vi "project.Industrial_Control.vi"() -> ()   [LabVIEW 2020]
doc: "ASTRA educational industrial automation simulation. Six-tab HMI; role-based authentication; conveyor state machine; deterministic sensors; alarm lifecycle; CSV journal. Logout/timeout/Exit request a controlled stop. No physical I/O or certified safety function. See docs/Engineering_Report.pdf and TEST_RESULTS.md. Public demonstration credentials only."
panel:
  out "Access level":string="None"
  out "Current operator":string="None"
  out "Authentication status":string="Signed out - enter your credentials"
  in  "Navigation":T1(tab)
  out "Can administer":bool
  out "Can acknowledge or reset":bool
  out "Can start or stop":bool
  out "Account lockout remaining (s)":dbl
  in  "Logout":bool
  in  "Username":string
  in  "Password":string
  in  "Login":bool
  out "Authenticated":bool
  out "Failed attempts":dbl
  out "Motor current (A)":dbl
  out "Motor temperature (C)":dbl=25.0 caption="Motor temperature (°C)"
  in  "Start conveyor":bool
  in  "Stop conveyor":bool
  out "Machine state":T2(ring)
  out "Operating mode":string="SOFTWARE SIMULATION"
  out "Motor speed (RPM)":dbl(knob) scale=0.0..1500.0
  out "Motor running":bool
  out "Motor stopped":bool=TRUE
  out "Machine fault":bool
  out "Machine message":string="Initializing"
  out "Sensor quality":string="GOOD"
  out "Monitoring trip":bool
  out "Current warning":bool
  out "Temperature warning":bool
  out "Sensor data valid":bool=TRUE
  out "Active current trip (A)":dbl=9.0
  out "Active current warning (A)":dbl=6.0
  out "Active temperature trip (C)":dbl=90.0 caption="Active temperature trip (°C)"
  out "Active temperature warning (C)":dbl=75.0 caption="Active temperature warning (°C)"
  out "Monitored speed (RPM)":dbl
  out "Current (A)":dbl(knob) scale=0.0..16.0
  out "Temperature (C)":dbl(knob)=25.0 caption="Temperature (°C)" scale=0.0..120.0
  out "Alarm history":string
  out "Unacknowledged alarms":dbl
  out "Active alarm severity":string="NORMAL"
  in  "Acknowledge all alarms":bool
  out "Alarm register":string[][](table)
  in  "Reset fault":bool
  out "Audit history":string
  out "CSV log path":path=path "logs/events.csv"
  in  "Inject sensor failure":bool
  in  "Inject overtemperature":bool
  in  "Apply monitoring settings":bool
  in  "Current trip setpoint (A)":dbl=9.0
  in  "Current warning setpoint (A)":dbl=6.0
  in  "Temperature trip setpoint (C)":dbl=90.0 caption="Temperature trip setpoint (°C)"
  in  "Temperature warning setpoint (C)":dbl=75.0 caption="Temperature warning setpoint (°C)"
  in  "Start permissive healthy":bool=TRUE
  in  "Inject motor overload":bool
  in  "Inject drive fault":bool
  in  "Generate demo password":bool
  out "Generated demonstration password":string
  out "Settings result":string="Default thresholds active"
  out "Session remaining (s)":dbl
  out "Audit write healthy":bool=TRUE
  in  "Exit application":bool
  # "INDUSTRIAL CONTROL & MONITORING"
  # "Credentials are case-sensitive. Three failures lock that account for 30 seconds."
  # "Use the demonstration account details in README.md. Logout before changing users."
  # "Logout / timeout: controlled stop. Fault reset: Maintenance or Administrator."
  # "Only Administrators can change simulation inputs and thresholds."
  # "ADMINISTRATOR UTILITY"
  # "This utility does not create, replace or reveal an authentication password."
  # "Ordinary random numbers are not cryptographically secure. Output is never logged."
  # "The original ten-iteration For Loop is retained with corrected digit conversion."
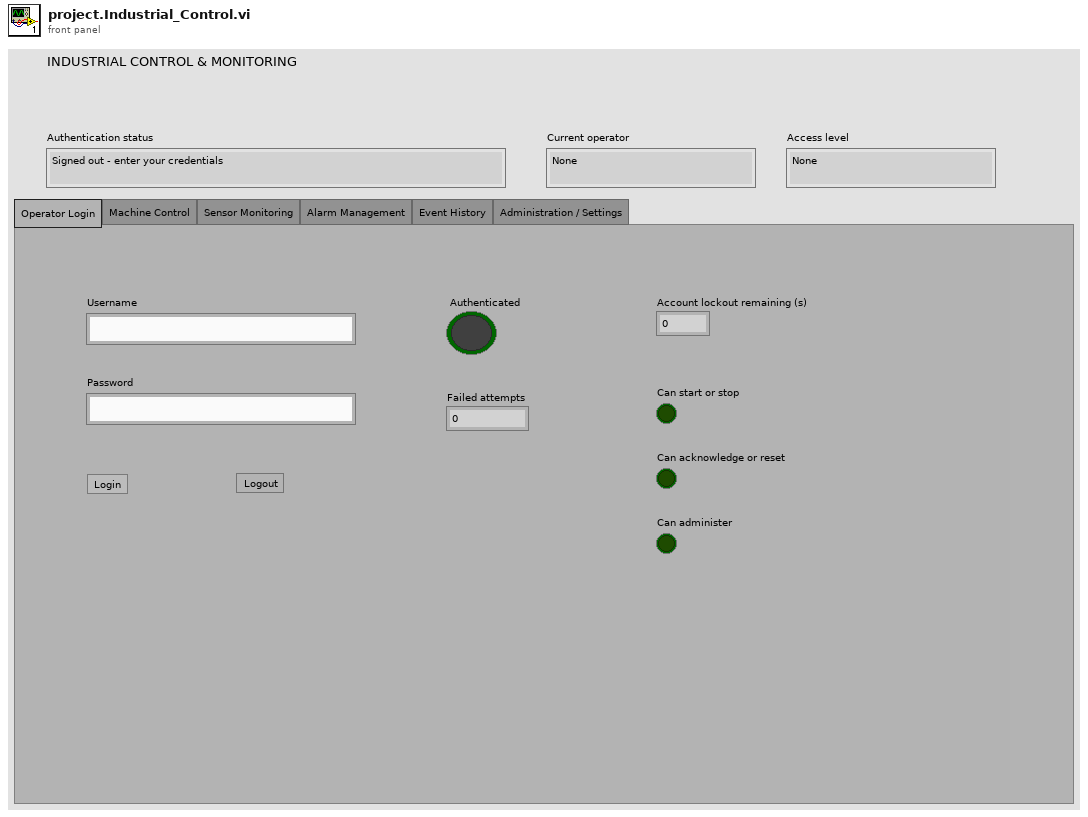
[diagram p1: front panel]
types:
  T1 = enum32{"Operator Login", "Machine Control", "Sensor Monitoring", "Alarm Management", "Event History", "Administration / Settings"}
  T2 = enum16{"INITIALIZATION", "IDLE", "READY", "RUNNING", "STOPPING", "FAULT", "RESETTING"}
  T3 = cluster{"A101":string, "A102":string, "A103":string, "A104":string, "A105":string, "A106":string, "A107":string, "A108":string, "A109":string}
  T4 = cluster{"A101 Active":dbl, "A101 Acknowledged":dbl, "A101 Seen":dbl, "A101 Changed":dbl, "A102 Active":dbl, "A102 Acknowledged":dbl, "A102 Seen":dbl, "A102 Changed":dbl, "A103 Active":dbl, "A103 Acknowledged":dbl, "A103 Seen":dbl, "A103 Changed":dbl, "A104 Active":dbl, "A104 Acknowledged":dbl, "A104 Seen":dbl, "A104 Changed":dbl, "A105 Active":dbl, "A105 Acknowledged":dbl, "A105 Seen":dbl, "A105 Changed":dbl, "A106 Active":dbl, "A106 Acknowledged":dbl, "A106 Seen":dbl, "A106 Changed":dbl, "A107 Active":dbl, "A107 Acknowledged":dbl, "A107 Seen":dbl, "A107 Changed":dbl, "A108 Active":dbl, "A108 Acknowledged":dbl, "A108 Seen":dbl, "A108 Changed":dbl, "A109 Active":dbl, "A109 Acknowledged":dbl, "A109 Seen":dbl, "A109 Changed":dbl}
  T5 = cluster{"Temperature C":dbl, "Current A":dbl, "Previous tick ms":dbl, "Temperature warning C":dbl, "Temperature trip C":dbl, "Current warning A":dbl, "Current trip A":dbl, "Settings result":dbl}
  T6 = cluster{"Machine state":enum16{"INITIALIZATION", "IDLE", "READY", "RUNNING", "STOPPING", "FAULT", "RESETTING"}, "Speed RPM":dbl, "Previous tick ms":dbl, "Reset started ms":dbl, "Latched fault code":dbl, "Command result":dbl, "Transition sequence":dbl}
  T7 = cluster{"Operator failures":dbl, "Maintenance failures":dbl, "Administrator failures":dbl, "Operator lock start ms":dbl, "Maintenance lock start ms":dbl, "Administrator lock start ms":dbl, "Active account":dbl, "Last activity ms":dbl, "Status code":dbl, "Event sequence":dbl}
  T8 = cluster{"Machine state":enum16{"INITIALIZATION", "IDLE", "READY", "RUNNING", "STOPPING", "FAULT", "RESETTING"}, "Speed RPM":dbl, i16, i16, i16, i16, i16, "Temperature warning setpoint (C)":dbl, "Temperature trip setpoint (C)":dbl, "Current warning setpoint (A)":dbl, "Current trip setpoint (A)":dbl}
  T9 = cluster{"High temperature warning":dbl, "Overtemperature trip":dbl, "High current warning":dbl, "Overload trip":dbl, "Sensor failure":dbl}
  T10 = cluster{"High temperature warning":dbl, "Overtemperature trip":dbl, "High current warning":dbl, "Overload trip":dbl, "Sensor failure":dbl, "unauthorized":dbl, "locked":dbl, i16, "permit_alarm":dbl}
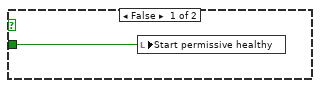
[diagram p2: hidden frame]
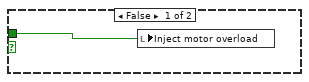
[diagram p3: hidden frame]
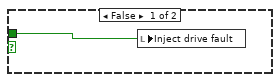
[diagram p4: hidden frame]
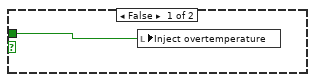
[diagram p5: hidden frame]
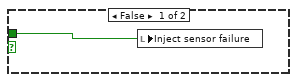
[diagram p6: hidden frame]
diagram:
  n1 = control-ref of="This VI"() -> (w23:refnum<vi>)
  n2 = property class="VI"(reference=w23) -> ("Path"=w22:path)  [unwired: 1 in, 2 out]
  n3 = Strip Path(path=w22) -> (stripped path=w21:path)  [unwired: 1 out]
  n4 = Build Path(base path=w21, name or relative path="logs\\events.csv") -> (appended path=w19:path)
  n5 = while {
    shift-right: [w446] -> _
    shift-left: T7 {"Operator failures"=0.0, "Maintenance failures"=0.0, "Administrator failures"=0.0, "Operator lock start ms"=-1.0, "Maintenance lock start ms"=-1.0, "Administrator lock start ms"=-1.0, "Active account"=-1.0, "Last activity ms"=0.0, "Status code"=0.0, "Event sequence"=0.0} ("State in") -> [w445]
    shift-right: ["Username"] -> _
    shift-left: "" -> [w439]
    shift-right: ["Password"] -> _
    shift-left: "" -> [w438]
    shift-right: ["Navigation"] -> _
    shift-left: 0 -> [w434]
    shift-right: [w390] -> _
    shift-left: "" -> [w391]
    tunnel: w19 -> [w382]
    tunnel: w19 -> [_]
    shift-right: [w381] -> _
    shift-left: "" -> [w380]
    shift-right: [w379] -> _
    shift-left: TRUE -> [w378]
    shift-right: [w377] -> _
    shift-left: T6 {"Machine state"=enum."INITIALIZATION", "Speed RPM"=0.0, "Previous tick ms"=-1.0, "Reset started ms"=-1.0, "Latched fault code"=0.0, "Command result"=0.0, "Transition sequence"=0.0} ("State in") -> [w376]
    shift-right: [w371] -> _
    shift-left: FALSE -> [w372]
    shift-right: [w29] -> _
    shift-left: TRUE -> [w359]
    shift-right: [w30] -> _
    shift-left: FALSE -> [w354]
    shift-right: [w31] -> _
    shift-left: FALSE -> [w349]
    shift-right: ["Start permissive healthy"] -> _
    shift-left: TRUE -> [w332]
    shift-right: ["Inject motor overload"] -> _
    shift-left: FALSE -> [w329]
    shift-right: ["Inject drive fault"] -> _
    shift-left: FALSE -> [w326]
    shift-right: [w32] -> _
    shift-left: FALSE -> [w274]
    shift-right: [w33] -> _
    shift-left: FALSE -> [w269]
    shift-right: [w247] -> _
    shift-left: T5 {"Temperature C"=25.0, "Current A"=0.0, "Previous tick ms"=-1.0, "Temperature warning C"=75.0, "Temperature trip C"=90.0, "Current warning A"=6.0, "Current trip A"=9.0, "Settings result"=0.0} ("State in") -> [w246]
    shift-right: [w188] -> _
    shift-left: T4 {"A101 Active"=0.0, "A101 Acknowledged"=1.0, "A101 Seen"=0.0, "A101 Changed"=0.0, "A102 Active"=0.0, "A102 Acknowledged"=1.0, "A102 Seen"=0.0, "A102 Changed"=0.0, "A103 Active"=0.0, "A103 Acknowledged"=1.0, "A103 Seen"=0.0, "A103 Changed"=0.0, "A104 Active"=0.0, "A104 Acknowledged"=1.0, "A104 Seen"=0.0, "A104 Changed"=0.0, "A105 Active"=0.0, "A105 Acknowledged"=1.0, "A105 Seen"=0.0, "A105 Changed"=0.0, "A106 Active"=0.0, "A106 Acknowledged"=1.0, "A106 Seen"=0.0, "A106 Changed"=0.0, "A107 Active"=0.0, "A107 Acknowledged"=1.0, "A107 Seen"=0.0, "A107 Changed"=0.0, "A108 Active"=0.0, "A108 Acknowledged"=1.0, "A108 Seen"=0.0, "A108 Changed"=0.0, "A109 Active"=0.0, "A109 Acknowledged"=1.0, "A109 Seen"=0.0, "A109 Changed"=0.0} ("State in") -> [w187]
    shift-right: [w158] -> _
    shift-left: T3 {"A101"="", "A102"="", "A103"="", "A104"="", "A105"="", "A106"="", "A107"="", "A108"="", "A109"=""} ("Previous timestamps") -> [w157]
    shift-right: [w149] -> _
    shift-left: "" -> [w151]
    shift-right: ["Inject overtemperature"] -> _
    shift-left: FALSE -> [w49]
    shift-right: ["Inject sensor failure"] -> _
    shift-left: FALSE -> [w46]
    stop <- w333 stop-if-true
    w115 = ""
    (unwired) "\t"
    w162 = "system"
    n6 = Wait (ms)(milliseconds to wait=50) -> ()  [unwired: 1 out]
    n7 = Select(t=1, s="Start conveyor", f=0) -> (s? t:f=w364:i32)
    n8 = Select(t=3, s="Reset fault", f=w364) -> (s? t:f=w361:i32)
    n9 = Select(t=3, s="Generate demo password", f=0) -> (s? t:f=w452:i32)
    n10 = Select(t=2, s="Stop conveyor", f=w361) -> (s? t:f=w340:i32)
    n11 = Not Equal?(x=w439, y="Username") -> (x != y?=w437:bool)
    n12 = Not Equal?(x=w438, y="Password") -> (x != y?=w436:bool)
    n13 = call "Final Demo Credential Lookup.vi"("Password"="Password", "Username"="Username") -> ("Credentials match"=w460:bool, "Account index"=w461:dbl)  [unwired: 8 in]
    n14 = Not Equal?(x=w332, y="Start permissive healthy") -> (x != y?=w330:bool)
    n15 = Or(x="Exit application", y="Logout") -> (x .or. y?=w450:bool)
    n16 = Not Equal To 0?(x=w340) -> (x != 0?=w331:bool)
    n17 = Select(t=1, s="Login", f=w452) -> (s? t:f=w448:i32)
    n18 = Or(x=w331, y=w330) -> (x .or. y?=w328:bool)
    n19 = Or(x=w436, y=w437) -> (x .or. y?=w433:bool)
    n20 = Not Equal?(x=w434, y="Navigation") -> (x != y?=w432:bool)
    n21 = Not Equal?(x=w329, y="Inject motor overload") -> (x != y?=w327:bool)
    n22 = Select(t=2, s=w450, f=w448) -> (s? t:f=w447:i32)
    n23 = Or(x=w328, y=w327) -> (x .or. y?=w325:bool)
    n24 = Or(x=w432, y=w433) -> (x .or. y?=w431:bool)
    n25 = Not Equal?(x=w326, y="Inject drive fault") -> (x != y?=w324:bool)
    n26 = Or(x="Acknowledge all alarms", y="Apply monitoring settings") -> (x .or. y?=w48:bool)
    n27 = Not Equal?(x=w49, y="Inject overtemperature") -> (x != y?=w47:bool)
    n28 = Not Equal To 0?(x=w447) -> (x != 0?=w430:bool)
    n29 = Or(x=w325, y=w324) -> (x .or. y?=w322:bool)
    n30 = Or(x=w430, y=w431) -> (x .or. y?=w429:bool)
    n31 = Not Equal?(x=w46, y="Inject sensor failure") -> (x != y?=w44:bool)
    n32 = Or(x=w48, y=w47) -> (x .or. y?=w45:bool)
    n33 = Or(x=w45, y=w44) -> (x .or. y?=w42:bool)
    n34 = Boolean To (0,1)(Boolean=w322) -> (0, 1=w321:i16)
    n35 = Boolean To (0,1)(Boolean=w429) -> (0, 1=w323:i16)
    n36 = Unbundle(w376) -> ("Machine state"=w244:T2, "Speed RPM"=w243:dbl)  [unwired: 5 out]
    n37 = Add(x=w323, y=w321) -> (x+y=w43:i16)
    n38 = Increment(x=w461) -> (x+1=w397:dbl)
    n39 = Boolean To (0,1)(Boolean=w460) -> (0, 1=w459:i16)
    n40 = Boolean To (0,1)(Boolean=w42) -> (0, 1=w41:i16)
    n41 = Boolean To (0,1)(Boolean="Apply monitoring settings") -> (0, 1=w239:i16)
    n42 = Boolean To (0,1)(Boolean="Apply monitoring settings") -> (0, 1=w196:i16)
    n43 = Add(x=w43, y=w41) -> (x+y=w40:i16)
    n44 = Tick Count (ms)() -> (millisecond timer value=w458:u32)
    n45 = call "Final Authentication Step.vi"("now"=w458, "user_activity"=w40, "password_ok"=w459, "account"=w461, "command"=w447, "State in"=w445) -> ("lock_seconds"=→"Account lockout remaining (s)":dbl, "actor"=w385:dbl, "event"=w384:dbl, "State out"=w446:T7, "generate"=w395:dbl, "session_seconds"=→"Session remaining (s)":dbl)
    n46 = Not Equal To 0?(x=w384) -> (x != 0?=w389:bool)
    n47 = Not Equal To 0?(x=w395) -> (x != 0?=w394:bool)
    n48 = Build Array("Signed out - enter your credentials", "Authenticated", "Invalid username or password", "Account locked for 30 seconds", "Login blocked - account lockout active", "Logged out", "Session expired - please log in again", "Access denied - administrator required", "Demo password generated", "Already logged in - log out before switching accounts") -> (w418:string[])
    n49 = Unbundle(w446) -> ("Operator failures"=w401:dbl, "Maintenance failures"=w400:dbl, "Administrator failures"=w399:dbl, "Active account"=w444:dbl, "Status code"=w417:dbl)  [unwired: 5 out]
    n50 = Unbundle(w446) -> ("Operator lock start ms"=w194:dbl, "Maintenance lock start ms"=w193:dbl, "Administrator lock start ms"=w192:dbl)  [unwired: 7 out]
    n51 = Build Array("None", "Operator", "Maintenance Technician", "Administrator") -> (w404:string[])
    n52 = case shown="True" w389 {
      frame False {
      }
      frame True {
        n53 = local write "Password"("") -> ()
      }
    }
    n54 = call "Final Check Permissions.vi"("Active account"=w444) -> ("Can administer"=w442:bool, "Can acknowledge or reset"=w443:bool, "Can start or stop"=w383:bool)  [unwired: 8 in]
    "Authenticated" <- w383
    "Can start or stop" <- w383
    "Can acknowledge or reset" <- w443
    "Can administer" <- w442
    n55 = case shown="True" w394 {
      tunnel: [w471 w472] -> w392
      tunnel: w391 -> [w471 _]
      frame False {
      }
      frame True {
        n56 = call "Final Generate Demo Password.vi"() -> ("Generated password"=w472:string)  [unwired: 11 in]
      }
    }
    n57 = Index Array(array=w418, index=w417) -> (element=→"Authentication status":string)
    n58 = Not Equal To 0?(x=w384) -> (x != 0?=w117:bool)
    n59 = Increment(x=w385) -> (x+1=w143:dbl)
    n60 = Increment(x=w444) -> (x+1=w410:dbl)
    n61 = Build Array(0, w401, w400, w399) -> (w398:dbl[])
    n62 = Index Array(array=w398, index=w397) -> (element=→"Failed attempts":dbl)
    n63 = Index Array(array=w404, index=w410) -> (element=→"Access level":string)
    n64 = Or(x=w372, y="Exit application") -> (x .or. y?=w371:bool)
    n65 = Not(x=w371) -> (.not. x?=w370:bool)
    n66 = And(x=w383, y=w370) -> (x .and. y?=w341:bool)
    n67 = Select(t="Inject drive fault", s=w442, f=w349) -> (s? t:f=w31:bool)
    n68 = Select(t="Start permissive healthy", s=w442, f=w359) -> (s? t:f=w29:bool)
    n69 = Select(t="Inject overtemperature", s=w442, f=w274) -> (s? t:f=w32:bool)
    n70 = Select(t="Inject sensor failure", s=w442, f=w269) -> (s? t:f=w33:bool)
    n71 = Select(t="Inject motor overload", s=w442, f=w354) -> (s? t:f=w30:bool)
    n72 = Select(t=0, s=w443, f=2) -> (s? t:f=w248:i32)
    n73 = Select(t=0, s=w443, f=2) -> (s? t:f=w291:i32)
    n74 = Select(t=0, s=w442, f=2) -> (s? t:f=w271:i32)
    n75 = Select(t=0, s=w442, f=2) -> (s? t:f=w356:i32)
    n76 = Select(t=0, s=w442, f=2) -> (s? t:f=w257:i32)
    n77 = Select(t=0, s=w442, f=2) -> (s? t:f=w260:i32)
    n78 = Select(t=0, s=w442, f=2) -> (s? t:f=w351:i32)
    n79 = Select(t=0, s=w442, f=2) -> (s? t:f=w346:i32)
    n80 = Select(t=0, s=w442, f=2) -> (s? t:f=w386:i32)
    n81 = Select(t=0, s=w442, f=2) -> (s? t:f=w266:i32)
    n82 = Select(t=0, s=w442, f=2) -> (s? t:f=w254:i32)
    n83 = Select(t=0, s=w442, f=2) -> (s? t:f=w251:i32)
    n84 = Select(t=0, s=w442, f=2) -> (s? t:f=w263:i32)
    n85 = property on="Acknowledge all alarms" class="Bool"("DisabledEnum"=w248) -> ()  [unwired: 2 in, 2 out]
    n86 = property on="Reset fault" class="Bool"("DisabledEnum"=w291) -> ()  [unwired: 2 in, 2 out]
    n87 = case shown="True" w442 {
      tunnel: w31 -> [w467 _]
      frame False {
        n88 = local write "Inject drive fault"(w467) -> ()
      }
      frame True {
      }
    }
    n89 = property on="Inject overtemperature" class="Bool (strict)"("DisabledEnum"=w271) -> ()  [unwired: 2 in, 2 out]
    n90 = case shown="True" w442 {
      tunnel: w30 -> [w466 _]
      frame False {
        n91 = local write "Inject motor overload"(w466) -> ()
      }
      frame True {
      }
    }
    n92 = case shown="True" w442 {
      tunnel: w32 -> [w468 _]
      frame False {
        n93 = local write "Inject overtemperature"(w468) -> ()
      }
      frame True {
      }
    }
    n94 = case shown="True" w442 {
      tunnel: w33 -> [w469 _]
      frame False {
        n95 = local write "Inject sensor failure"(w469) -> ()
      }
      frame True {
      }
    }
    n96 = property on="Start permissive healthy" class="Bool (strict)"("DisabledEnum"=w356) -> ()  [unwired: 2 in, 2 out]
    n97 = property on="Temperature trip setpoint (C)" class="DigNum (strict)"("DisabledEnum"=w257) -> ()  [unwired: 2 in, 2 out]
    n98 = case shown="True" w442 {
      tunnel: w29 -> [w465 _]
      frame False {
        n99 = local write "Start permissive healthy"(w465) -> ()
      }
      frame True {
      }
    }
    n100 = property on="Temperature warning setpoint (C)" class="DigNum (strict)"("DisabledEnum"=w260) -> ()  [unwired: 2 in, 2 out]
    n101 = property on="Inject motor overload" class="Bool (strict)"("DisabledEnum"=w351) -> ()  [unwired: 2 in, 2 out]
    n102 = property on="Inject drive fault" class="Bool (strict)"("DisabledEnum"=w346) -> ()  [unwired: 2 in, 2 out]
    n103 = property on="Generate demo password" class="Bool"("DisabledEnum"=w386) -> ()  [unwired: 2 in, 2 out]
    n104 = property on="Inject sensor failure" class="Bool (strict)"("DisabledEnum"=w266) -> ()  [unwired: 2 in, 2 out]
    n105 = property on="Current warning setpoint (A)" class="DigNum (strict)"("DisabledEnum"=w254) -> ()  [unwired: 2 in, 2 out]
    n106 = property on="Current trip setpoint (A)" class="DigNum (strict)"("DisabledEnum"=w251) -> ()  [unwired: 2 in, 2 out]
    n107 = property on="Apply monitoring settings" class="Bool"("DisabledEnum"=w263) -> ()  [unwired: 2 in, 2 out]
    n108 = Boolean To (0,1)(Boolean=w30) -> (0, 1=w242:i16)
    n109 = Boolean To (0,1)(Boolean=w32) -> (0, 1=w241:i16)
    n110 = Boolean To (0,1)(Boolean=w33) -> (0, 1=w240:i16)
    n111 = Boolean To (0,1)(Boolean=w442) -> (0, 1=w238:i16)
    n112 = Select(t=1, s=w30, f=0) -> (s? t:f=w342:i32)
    n113 = Bundle("Machine state"=w244, "Speed RPM"=w243, w242, w241, w240, w239, w238, "Temperature warning setpoint (C)"="Temperature warning setpoint (C)", "Temperature trip setpoint (C)"="Temperature trip setpoint (C)", "Current warning setpoint (A)"="Current warning setpoint (A)", "Current trip setpoint (A)"="Current trip setpoint (A)") -> (w233:T8)  [unwired: 1 in]
    n114 = Select(t=2, s=w31, f=w342) -> ()  [unwired: 1 out]
    n115 = call "Final Monitoring Step.vi"("Tick ms"=w458, "Inputs"=w233, "State in"=w246) -> ("Trip code"=w220:dbl, "Conditions"=w232:T9, "State out"=w247:T5)  [unwired: 6 in]
    n116 = Select(t=w392, s=w442, f="") -> (s? t:f=w390:string)
    "Generated demonstration password" <- w390
    n117 = Boolean To (0,1)(Boolean=w341) -> (0, 1=w339:i16)
    n118 = Boolean To (0,1)(Boolean=w443) -> (0, 1=w338:i16)
    n119 = Boolean To (0,1)(Boolean=w31) -> (0, 1=w182:i16)
    n120 = Boolean To (0,1)(Boolean=w29) -> (0, 1=w191:i16)
    n121 = Boolean To (0,1)(Boolean=w29) -> (0, 1=w337:i16)
    n122 = Boolean To (0,1)(Boolean=w442) -> (0, 1=w195:i16)
    n123 = Select(t=2, s=w31, f=0) -> (s? t:f=w202:i32)
    n124 = Not Equal To 0?(x=w220) -> (x != 0?=→"Monitoring trip":bool)
    n125 = Not Equal To 0?(x=w220) -> (x != 0?=w203:bool)
    n126 = Unbundle(w247) -> ("Temperature C"=→"Motor temperature (C)" →"Temperature (C)":dbl, "Current A"=→"Motor current (A)" →"Current (A)":dbl, "Temperature warning C"=→"Active temperature warning (C)":dbl, "Temperature trip C"=w228:dbl, "Current warning A"=→"Active current warning (A)":dbl, "Current trip A"=w226:dbl, "Settings result"=w207:dbl)  [unwired: 1 out]
    "Active temperature trip (C)" <- w228
    "Active current trip (A)" <- w226
    n127 = Build Array("Default thresholds active", "Settings applied", "Rejected: warning must be below trip; check limits", "Access denied - Administrator required") -> (w208:string[])
    n128 = formula code="tmax=TT+20; if(tmax<120) tmax=120; imax=IT+5; if(imax<16) imax=16;"("TT"=w228, "IT"=w226) -> ("tmax"=w36:dbl, "imax"=w34:dbl)
    n129 = Select(t=w220, s=w203, f=w202) -> (s? t:f=w201:dbl)
    n130 = Index Array(array=w208, index=w207) -> (element=→"Settings result":string)
    n131 = property on="Temperature (C)" class="Knob (strict)"() -> ("Scale"=w37:refnum<vi>)  [unwired: 2 in, 2 out]
    n132 = property on="Current (A)" class="Knob (strict)"() -> ("Scale"=w35:refnum<vi>)  [unwired: 2 in, 2 out]
    n133 = property class="RtryColScl"(reference=w37, "Maximum"=w36) -> ()  [unwired: 1 in, 2 out]
    n134 = property class="RtryColScl"(reference=w35, "Maximum"=w34) -> ()  [unwired: 1 in, 2 out]
    n135 = Bundle(w340, w339, w338, w337, "Trip code"=w201) -> (w336:cluster{i32, i16, i16, i16, "Trip code":dbl})  [unwired: 1 in]
    n136 = call "Final Conveyor Step.vi"("Tick ms"=w458, "Commands"=w336, "State in"=w376) -> ("State out"=w377:T6)  [unwired: 8 in]
    n137 = Build Array("None", "operator", "maintenance", "admin") -> (w411:string[])
    n138 = Build Array("NONE", "LOGIN_SUCCESS", "LOGIN_FAILURE", "ACCOUNT_LOCKOUT", "LOGIN_BLOCKED", "LOGOUT", "SESSION_TIMEOUT", "UNAUTHORIZED_OPERATION", "DEMO_PASSWORD_GENERATED", "LOGIN_REJECTED") -> (w132:string[])
    n139 = Build Array("State transition", "Start accepted", "Stop requested", "Reset accepted", "Access denied", "Start requires READY and healthy permissives", "Active or latched fault prevents operation", "No fault available to reset", "Reserved", "Motor must stop before reset") -> (w96:string[])
    n140 = Build Array("Ready for commands", "Start accepted", "Stop requested", "Reset accepted - checking clear conditions", "Access denied for this operation", "Start requires READY state and healthy permissives", "Active or latched fault prevents operation", "No fault is available to reset", "Reserved", "Wait until the motor is stopped before reset") -> (w303:string[])
    n141 = Build Array("INITIALIZATION", "IDLE", "READY", "RUNNING", "STOPPING", "FAULT", "RESETTING") -> (w107:string[])
    n142 = Build Array("INITIALIZATION", "IDLE", "READY", "RUNNING", "STOPPING", "FAULT", "RESETTING") -> (w163:string[])
    n143 = Build Array("Initializing", "Signed out or start permissive unavailable", "Ready to start", "Running", "Controlled stop in progress", "Fault latched - authorized reset required", "Resetting - verifying cleared fault") -> (w283:string[])
    n144 = Build Array("unknown/system", "operator", "maintenance", "admin") -> (w144:string[])
    n145 = Build Array("NONE", "SETTINGS_APPLIED", "SETTINGS_REJECTED", "UNAUTHORIZED_OPERATION") -> (w70:string[])
    n146 = Build Array("No change", "Validated monitoring thresholds applied", "Rejected invalid monitoring thresholds", "Unauthorized settings change rejected") -> (w65:string[])
    n147 = Index Array(array=w411, index=w410) -> (element=w409:string)
    "Current operator" <- w409
    n148 = Boolean To (0,1)(Boolean=w443) -> (0, 1=w197:i16)
    n149 = Unbundle(w377) -> ("Machine state"=w190:T2, "Speed RPM"=→"Monitored speed (RPM)":dbl, "Latched fault code"=w189:dbl, "Command result"=w199:dbl)  [unwired: 3 out]
    n150 = Boolean To (0,1)(Boolean="Acknowledge all alarms") -> (0, 1=w198:i16)
    n151 = Unbundle(w377) -> ("Machine state"=w375:T2, "Speed RPM"=w374:dbl, "Latched fault code"=w320:dbl, "Command result"=w302:dbl)  [unwired: 3 out]
    "Machine state" <- w375
    "Motor speed (RPM)" <- w374
    n152 = Build Array("", "Authenticated successfully", "Invalid username or password", "Third consecutive failure; locked for 30 seconds", "Login refused during account lockout", "Operator logged out", "Session expired after 60 seconds of inactivity", "Administrator permission required", "Ten-digit demonstration password generated; value omitted", "Log out before switching accounts") -> (w121:string[])
    n153 = Build Array("", "OVERLOAD TRIP - clear injection, stop, then authorized reset", "DRIVE FAULT - clear injection, stop, then authorized reset", "PERMISSIVE LOST - restore permissive, stop, then authorized reset", "OVERTEMPERATURE - cool below trip limit, then authorized reset", "SENSOR FAILURE - restore valid sensors, then authorized reset") -> (w297:string[])
    n154 = formula code="unauthorized=((command!=0 && result==4) || auth_event==7 || (ack!=0 && can_ack==0) || (apply!=0 && admin==0)); locked=(l0>=0 || l1>=0 || l2>=0); permit_alarm=(permit==0 && (state==3 || state==4 || fault==3));"("command"=w340, "result"=w199, "auth_event"=w384, "ack"=w198, "can_ack"=w197, "apply"=w196, "admin"=w195, "l0"=w194, "l1"=w193, "l2"=w192, "permit"=w191, "state"=w190, "fault"=w189) -> ("unauthorized"=w184:dbl, "locked"=w183:dbl, "permit_alarm"=w181:dbl)
    n155 = formula code="event=0;\nif(command!=0 && result==4) event=6;\nelse if(state!=previous) {\n if(state==3) event=1; else if(state==4) event=2; else if(state==5) event=3;\n else if(state==6) event=4; else if(previous==6) event=5; else event=9;\n} else if(command!=0) { if(result==5 || result==6 || result==7 || result==9) event=7; else event=8; }"("state"=w190, "previous"=w244, "command"=w340, "result"=w199) -> ("event"=w80:dbl)
    n156 = formula code="running=(state==3 && rpm>0); stopped=(rpm==0); faulted=(fault!=0);"("state"=w375, "rpm"=w374, "fault"=w320) -> ("running"=w319:dbl, "stopped"=w317:dbl, "faulted"=w315:dbl)
    n157 = Select(t="ALARM_ACKNOWLEDGMENT", s=w443, f="UNAUTHORIZED_OPERATION") -> (s? t:f=w57:string)
    n158 = Select(t="Acknowledge all alarms requested", s=w443, f="Unauthorized alarm acknowledgment rejected") -> (s? t:f=w56:string)
    n159 = Select(t=w409, s="Acknowledge all alarms", f=w162) -> (s? t:f=w160:string)
    n160 = Index Array(array=w121, index=w384) -> (element=w118:string)
    n161 = Index Array(array=w132, index=w384) -> (element=w119:string)
    n162 = Index Array(array=w144, index=w143) -> (element=w120:string)
    n163 = Index Array(array=w107, index=w244) -> (element=w95:string)
    n164 = Index Array(array=w70, index=w207) -> (element=w64:string)
    n165 = Index Array(array=w65, index=w207) -> (element=w63:string)
    n166 = Index Array(array=w96, index=w199) -> (element=w92:string)
    n167 = Index Array(array=w283, index=w375) -> (element=w281:string)
    n168 = Equal To 0?(x=w374) -> (x = 0?=w334:bool)
    n169 = Index Array(array=w297, index=w320) -> (element=w295:string)
    n170 = Select(t=w409, s=w383, f=w162) -> (s? t:f=w79:string)
    n171 = Index Array(array=w303, index=w302) -> (element=w294:string)
    n172 = Index Array(array=w163, index=w190) -> (element=w159:string)
    n173 = Not Equal To 0?(x=w320) -> (x != 0?=w296:bool)
    n174 = Not Equal To 0?(x=w302) -> (x != 0?=w282:bool)
    n175 = Unbundle(w232) -> ("High temperature warning"=w224:dbl, "Overtemperature trip"=w186:dbl, "High current warning"=w222:dbl, "Overload trip"=w185:dbl, "Sensor failure"=w218:dbl)
    n176 = Format Date/Time String(time format string (%c)="%Y-%m-%dT%H:%M:%SZ", UTC format=TRUE) -> (date/time string=w161:string)  [unwired: 1 in]
    n177 = Select(t=w295, s=w296, f=w294) -> ()  [unwired: 1 out]
    n178 = call "Final Format Event.vi"("Machine state"=w159, "Description"=w63, "Category"=w64, "Source"=w79, "Timestamp UTC"=w161) -> ("CSV record"=w62:string)  [unwired: 6 in]
    n179 = call "Final Format Event.vi"("Machine state"=w159, "Description"=w118, "Category"=w119, "Source"=w120, "Timestamp UTC"=w161) -> ("CSV record"=w116:string)  [unwired: 6 in]
    n180 = call "Final Format Event.vi"("Machine state"=w159, "Description"=w56, "Category"=w57, "Source"=w79, "Timestamp UTC"=w161) -> ("CSV record"=w55:string)  [unwired: 6 in]
    n181 = And(x=w371, y=w334) -> (x .and. y?=w333:bool)
    n182 = Build Array("NONE", "MACHINE_START", "MACHINE_STOP", "MACHINE_TRIP", "FAULT_RESET_REQUEST", "FAULT_RESET_COMPLETE", "UNAUTHORIZED_OPERATION", "MACHINE_COMMAND_REJECTED", "MACHINE_COMMAND", "MACHINE_STATE") -> (w81:string[])
    n183 = Bundle("High temperature warning"=w224, "Overtemperature trip"=w186, "High current warning"=w222, "Overload trip"=w185, "Sensor failure"=w218, "unauthorized"=w184, "locked"=w183, w182, "permit_alarm"=w181) -> (w180:T10)  [unwired: 1 in]
    n184 = Not Equal To 0?(x=w224) -> (x != 0?=→"Temperature warning":bool)
    n185 = Not Equal To 0?(x=w222) -> (x != 0?=→"Current warning":bool)
    n186 = Not Equal To 0?(x=w319) -> (x != 0?=→"Motor running":bool)
    n187 = Not Equal To 0?(x=w317) -> (x != 0?=→"Motor stopped":bool)
    n188 = Not Equal To 0?(x=w315) -> (x != 0?=→"Machine fault":bool)
    n189 = Select(t=w294, s=w282, f=w281) -> (s? t:f=w280:string)
    n190 = Not Equal To 0?(x=w218) -> (x != 0?=w217:bool)
    n191 = Select(t=w295, s=w296, f=w280) -> ()  [unwired: 1 out]
    n192 = call "Final Alarm Step.vi"("Can acknowledge"=w197, "Acknowledge all"=w198, "Conditions"=w180, "State in"=w187) -> ("Unacknowledged count"=→"Unacknowledged alarms":dbl, "Active severity"=w174:dbl, "State out"=w188:T4)  [unwired: 5 in]
    n193 = Concatenate Strings(w95, " -> ", w159, "; ", w92) -> (w77:string)
    n194 = Concatenate Strings(w294, "\n", w295) -> (w278:string)
    n195 = Index Array(array=w81, index=w80) -> (element=w78:string)
    n196 = Not(x=w217) -> (.not. x?=→"Sensor data valid":bool)
    n197 = call "Final Format Event.vi"("Machine state"=w159, "Description"=w77, "Category"=w78, "Source"=w79, "Timestamp UTC"=w161) -> ("CSV record"=w75:string)  [unwired: 6 in]
    n198 = Select(t="BAD - readings held", s=w217, f="GOOD") -> (s? t:f=→"Sensor quality":string)
    n199 = Select(t=w278, s=w282, f=w295) -> (s? t:f=w277:string)
    n200 = Build Array("NORMAL", "WARNING", "TRIP") -> (w175:string[])
    n201 = Select(t=w62, s="Apply monitoring settings", f=w115) -> (s? t:f=w52:string)
    n202 = Select(t=w116, s=w117, f=w115) -> (s? t:f=w54:string)
    n203 = Select(t=w55, s="Acknowledge all alarms", f=w115) -> (s? t:f=w51:string)
    n204 = Select(t=w277, s=w296, f=w280) -> (s? t:f=→"Machine message":string)
    n205 = call "Final Format Alarm Register.vi"("Machine state"=w159, "Source"=w160, "Timestamp UTC"=w161, "Previous timestamps"=w157, "Alarm state"=w188) -> ("Alarm events"=w150:string, "Alarm register"=w156:string, "Timestamps out"=w158:T3)  [unwired: 4 in]
    n206 = Index Array(array=w175, index=w174) -> (element=→"Active alarm severity":string)
    n207 = Not Equal To 0?(x=w80) -> (x != 0?=w76:bool)
    n208 = Select(t=w75, s=w76, f=w115) -> (s? t:f=w53:string)
    n209 = call "Final History Tail.vi"("New records"=w150, "Previous history"=w151) -> ("Recent history"=w149:string)  [unwired: 9 in]
    "Alarm history" <- w149
    n210 = Concatenate Strings(w54, w53, w150, w52, w51) -> (w50:string)
    n211 = call "Final Event Journal.vi"("Previous write healthy"=w378, "Previous history"=w380, "Records"=w50, "CSV path"=w382) -> ("Write healthy"=w379:bool, "Recent history"=w381:string)  [unwired: 6 in]
    n212 = Spreadsheet String To Array(delimiter (Tab)="\t", format string="%s", spreadsheet string=w156, array type (2D Dbl)=string[][] [] ("Alarm register")) -> (array=→"Alarm register":string[][])
    "Audit history" <- w380
    "CSV log path" <- w382
    "Audit write healthy" <- w378
    "Operating mode" <- "SOFTWARE SIMULATION"
  }
